vi "DO NOT DELETE acps project main ().vi"() -> ()   [LabVIEW 2026]
uses:
  <vilib>/DAQmx/write.llb/DAQmx Write (Counter Frequency 1Chan 1Samp).vi
  <vilib>/DAQmx/create/channels.llb/DAQmx Create Channel (CO-Pulse Generation-Frequency).vi
  <vilib>/DAQmx/configure/timing.llb/DAQmx Timing (Implicit).vi
  <vilib>/DAQmx/miscellaneous.llb/DAQmx Fill In Error Info.vi
panel:
  in  "stop 3":bool
  out "vibrating motor / LDR":bool
  out "smoke":bool
  out "temperature":dbl
  out "humidity":dbl
  in  "Tab Control":enum32{"Overview", "Detailed", "Advanced"}(tab)
  in  "Tol":dbl=10.0
  in  "Reset":bool
  out "Rotation":bool
  out "Jars Filled":dbl
  out "Weight":dbl(slide) scale=0.0..200.0
  out "State":dbl(ring) items=["0: Indexing / Seeking Jar"=0.0, "1: Reading Jar Colour"=1.0, "2: Stage 1 Filling"=2.0, "3: Stage 2 Dumping"=3.0, "4: Settle & Count"=4.0, "5: Clearing IR Beam"=5.0, "9: FAULT LATCHED!"=9.0]
  out "Total Weights Filled":dbl
  out "Target Weight":dbl
  out "Grains filling":bool
  in  "Red Weight":dbl=100.0
  in  "Green Weight":dbl=200.0
  in  "Blue Weight":dbl=300.0
  in  "Tare\nTare\nt\nT":bool
  in  "stop":bool
  out "IR":dbl
  out "LDR":dbl
  out "level":bool
  out "?":dbl[](array[numeric])
  out "Waveform Chart":dbl(graph)
  out "Faults":dbl
  out "IR":dynamicdata(graph)
  out "ldr":dynamicdata(graph)
  in  "K for":dbl=1046000.0
  out "Spread":dbl
  out "Vm":dbl
  out "Stable":bool
  out "Allow":dbl
  out "cmt":dbl
  out "v0":dbl
  out "done":dbl
  in  "stop 2":bool
  out "max value for colour sensor":dbl(graph)
  out "col":i32
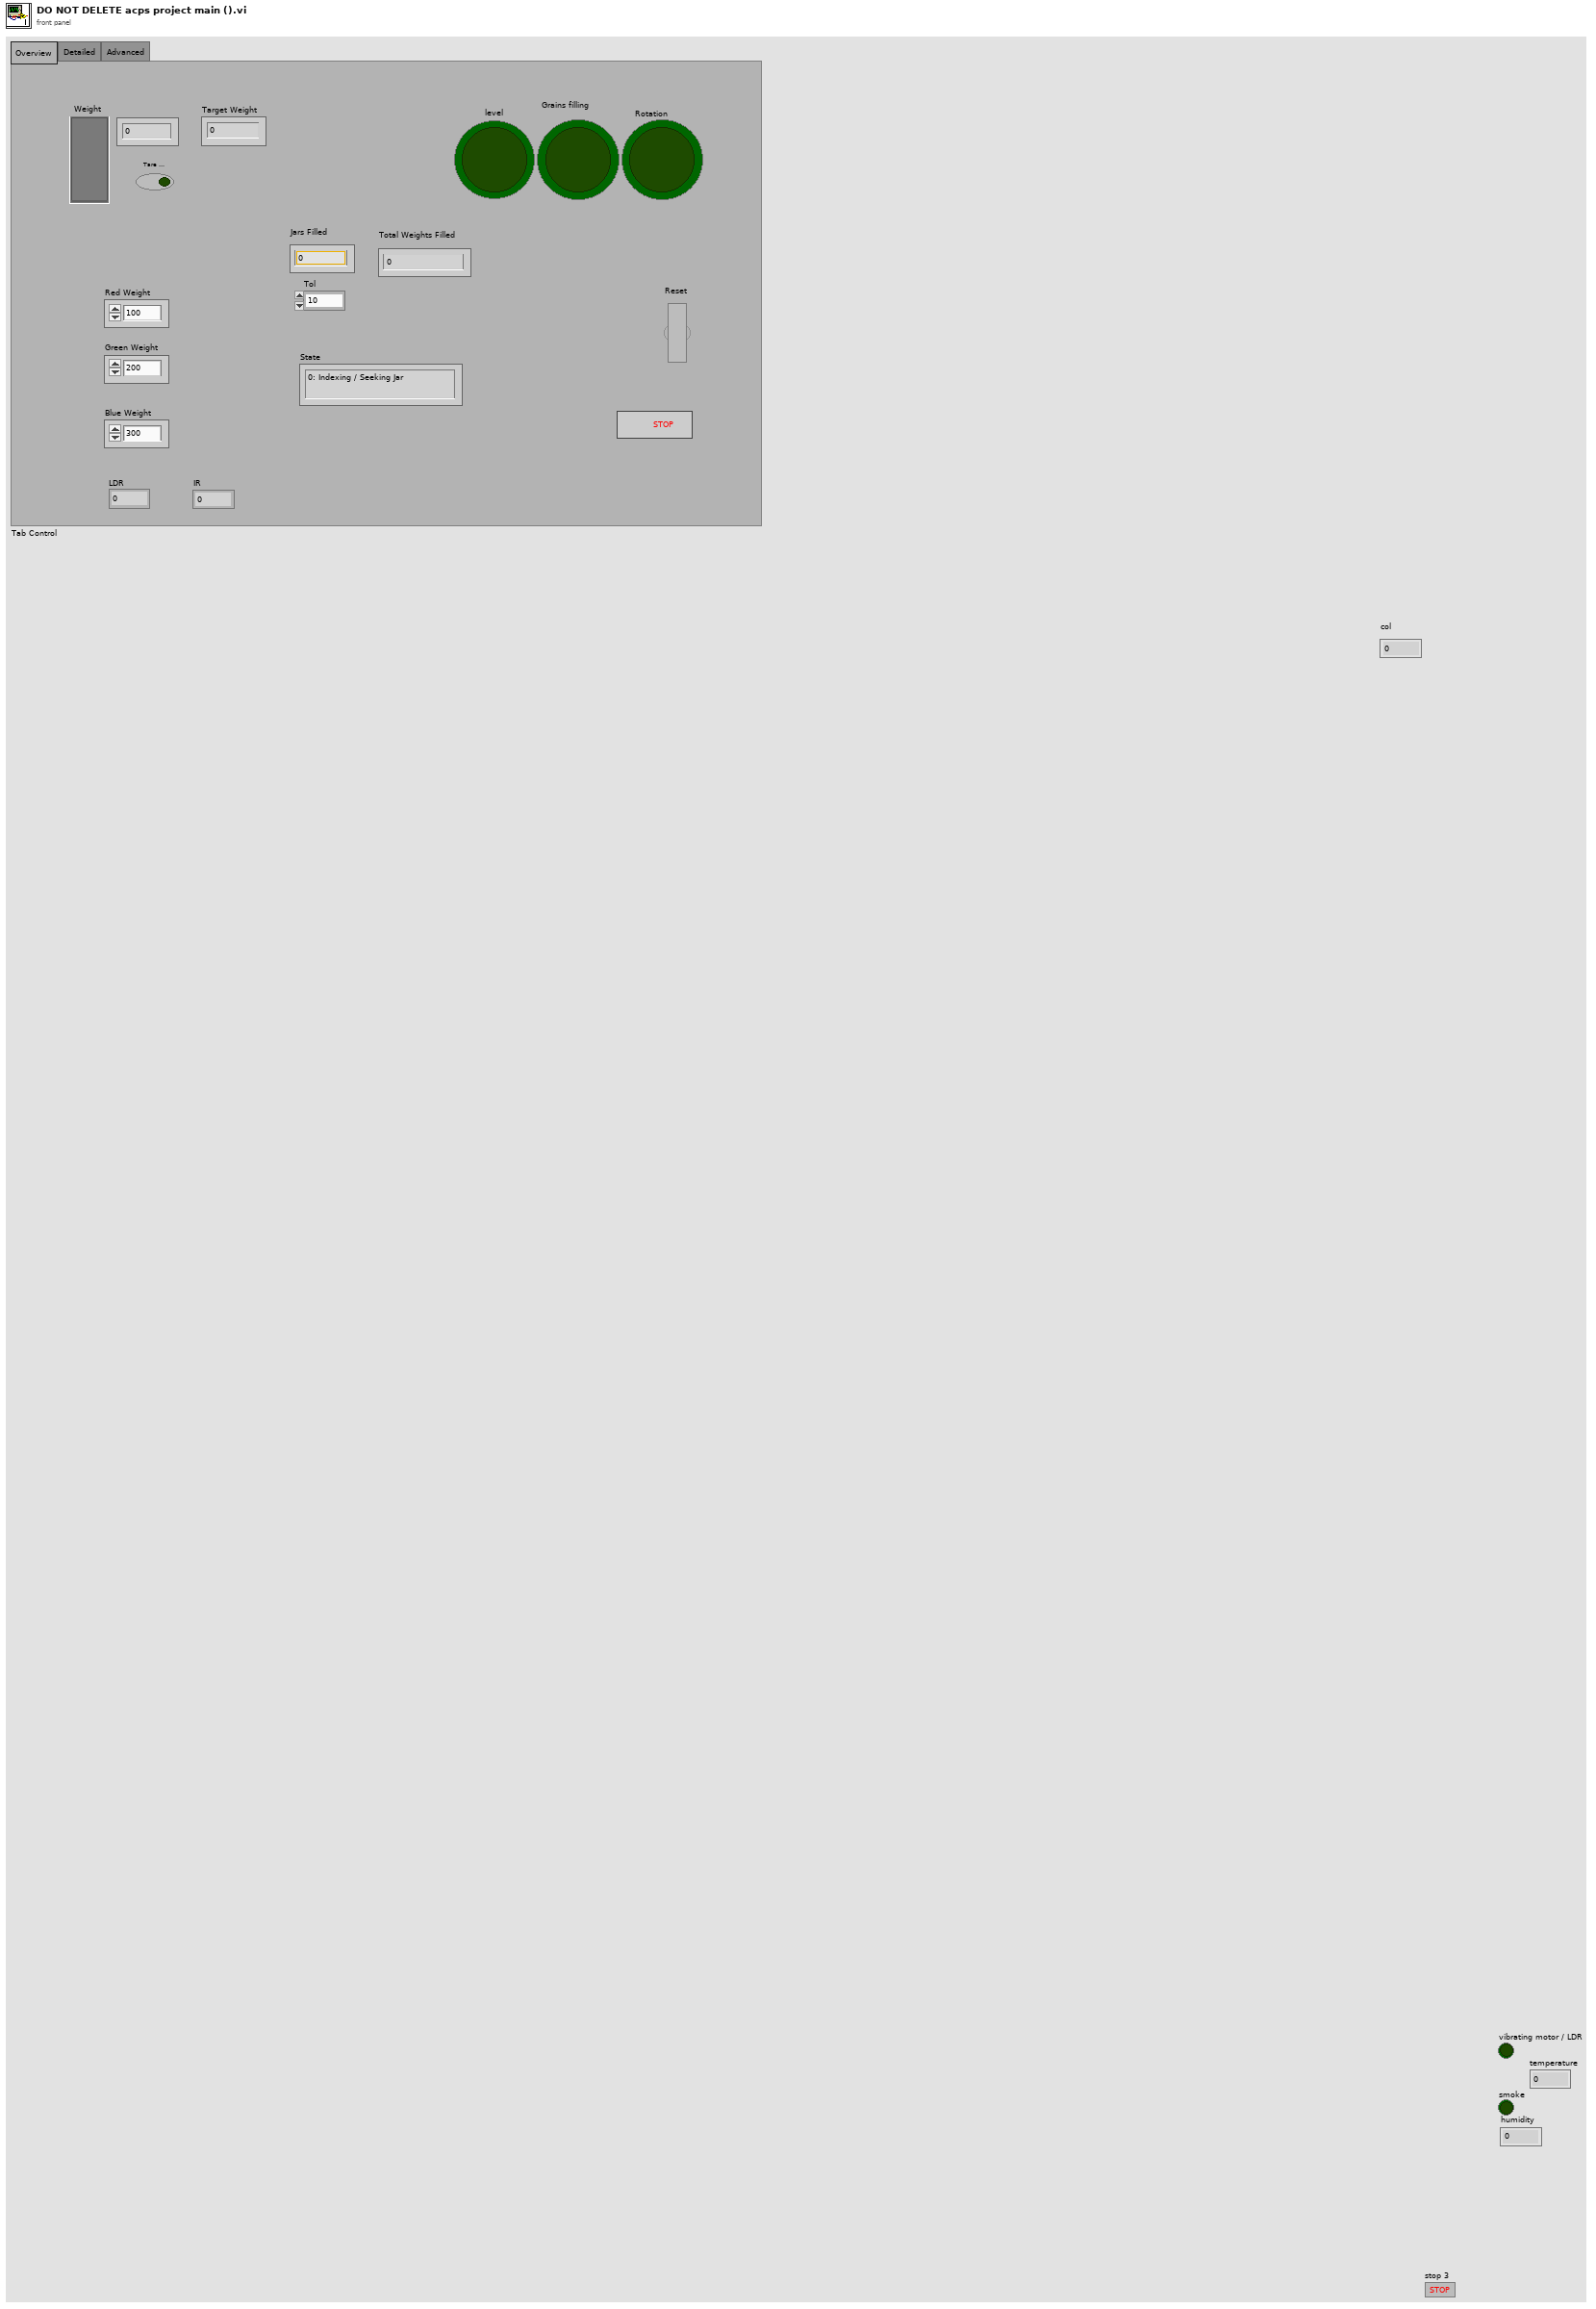
[diagram p1: front panel]
types:
  T1 = cluster{"LDR/Vibration ip":bool, "weight":dbl, "colour":i32}
  T2 = cluster{"vibrating motor / LDR":bool, "level sensor":bool, "Smoke/Fire":bool, "temperature":dbl, "humidity":dbl}
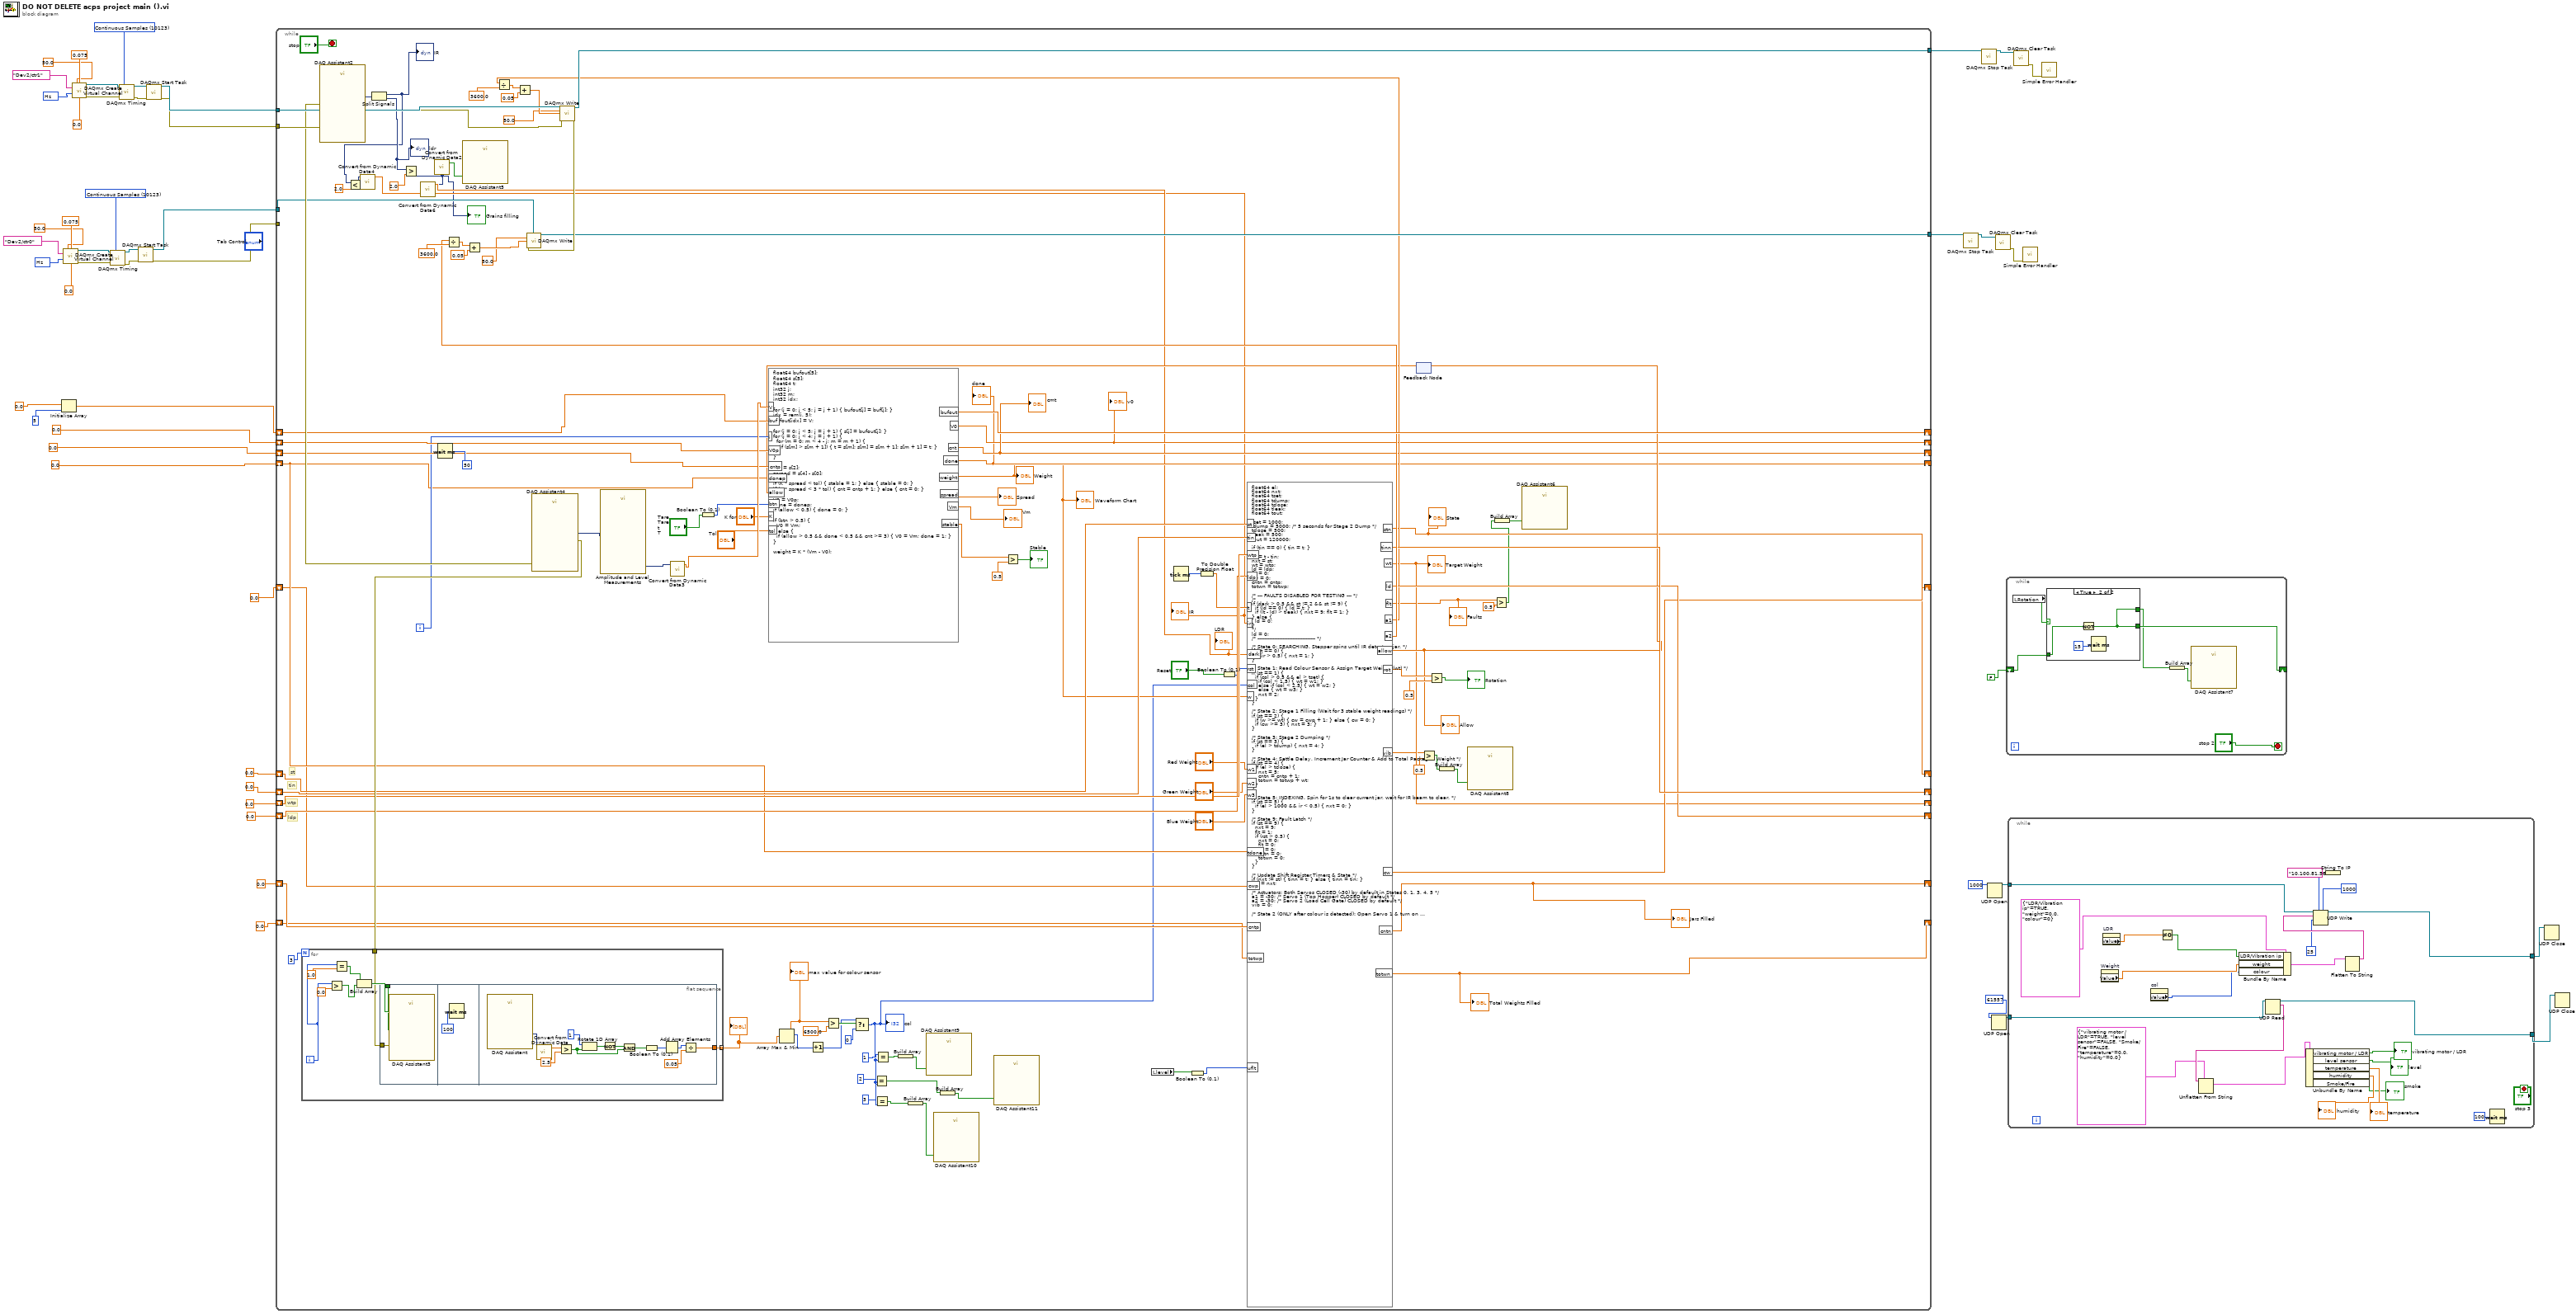
[diagram p0: block diagram]
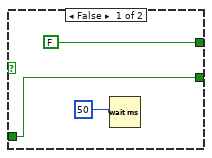
[diagram p2: hidden frame]
diagram:
  w25 = 10123 items=["Finite Samples"=10178, "Continuous Samples"=10123, "Hardware Timed Single Point"=12522] ("sample mode")
  w30 = 10373 items=["Hz"=10373] ("units")
  w45 = 10123 items=["Finite Samples"=10178, "Continuous Samples"=10123, "Hardware Timed Single Point"=12522] ("sample mode")
  w50 = 10373 items=["Hz"=10373] ("units")
  n1 = Initialize Array(0.0 ("element"), 5 ("dimension size")) -> (w10:dbl[])
  n2 = call-poly <vilib>:"DAQmx Create Virtual Channel.vi"("frequency"=50.0, "duty cycle"=0.075, "counter"=tag "Dev2/ctr0", "units"=w30, "initial delay"=0.0) -> ("task out"=w24:refnum<k21>, "error out"=w22:errorcluster)  [unwired: 9 in]
  n3 = call-poly <vilib>:"DAQmx Create Virtual Channel.vi"("frequency"=50.0, "duty cycle"=0.075, "counter"=tag "Dev2/ctr1", "units"=w50, "initial delay"=0.0) -> ("task out"=w44:refnum<k21>, "error out"=w41:errorcluster)  [unwired: 9 in]
  n4 = call-poly <vilib>:"DAQmx Timing.vi"("task/channels in"=w24, "sample mode"=w25, "error in"=w22) -> ("task out"=w23:refnum<k21>, "error out"=w21:errorcluster)  [unwired: 11 in]
  n5 = call-poly <vilib>:"DAQmx Timing.vi"("task/channels in"=w44, "sample mode"=w45, "error in"=w41) -> ("task out"=w43:refnum<k21>, "error out"=w40:errorcluster)  [unwired: 11 in]
  n6 = call <vilib>:"DAQmx Start Task.vi"("task/channels in"=w23, "error in"=w21) -> ("task out"=w20:refnum<k21>, "error out"=w19:errorcluster)  [unwired: 12 in]
  n7 = call <vilib>:"DAQmx Start Task.vi"("task/channels in"=w43, "error in"=w40) -> ("task out"=w42:refnum<k21>, "error out"=w39:errorcluster)  [unwired: 12 in]
  n8 = while {
    tunnel: w42 -> [w154]
    tunnel: w39 -> [w151]
    tunnel: [w149] -> w38
    shift-right: [w128] -> _
    shift-left: w10 -> [w137]
    shift-right: [w91] -> _
    shift-left: 0.0 ("element") -> [w90]
    shift-right: [w92] -> _
    shift-left: 0.0 ("element") -> [w136]
    shift-right: [w93] -> _
    shift-left: 0.0 ("element") -> [w135]
    tunnel: w20 -> [w122]
    tunnel: w19 -> [_]
    tunnel: [w120] -> w16
    shift-right: [w76] -> _
    shift-left: 0.0 -> [w113]
    shift-right: [w109] -> _
    shift-left: 0.0 -> [w112]
    shift-right: [w77] -> _
    shift-left: 0.0 -> [w111]
    shift-right: [w108] -> _
    shift-left: 0.0 -> [w110]
    shift-right: [w88] -> _
    shift-left: 0.0 -> [w89]
    shift-right: [w75] -> _
    shift-left: 0.0 -> [w83]
    shift-right: [w65] -> _
    shift-left: 0.0 -> [w66]
    i -> [w129]
    stop <- "stop" stop-if-true
    # "ldp"
    # "wtp"
    # "tin"
    # "st"
    n9 = call "DAQ Assistant2"() -> ("data"=w147:dynamicdata, "error out"=w145:errorcluster)  [unwired: 17 in, 1 out]
    n10 = Split Signals(w147) -> (w86:dynamicdata, w100:dynamicdata)  [unwired: 2 in]
    "IR" <- w86
    "ldr" <- w100
    n11 = Less?(x=w86, y=2.0) -> (x < y?=w85:dynamicdata)
    n12 = call "Convert from Dynamic Data4"("Dynamic Data Type"=w85) -> ("Scalar"=w79:dbl)  [unwired: 3 in]
    "IR" <- w79
    n13 = Greater?(x=w100, y=2.0) -> (0:w63:dynamicdata)
    "Grains filling" <- w63
    n14 = call "Convert from Dynamic Data6"("Dynamic Data Type"=w63) -> ("Scalar"=w80:dbl)  [unwired: 3 in]
    "LDR" <- w80
    n15 = call "Convert from Dynamic Data2"("Dynamic Data Type"=w63) -> ("Array"=w64:bool[])  [unwired: 3 in]
    n16 = Wait (ms)(milliseconds to wait=u32 50) -> ()  [unwired: 1 out]
    n17 = call "DAQ Assistant5"("data"=w64) -> ()  [unwired: 17 in, 2 out]
    n18 = call "DAQ Assistant4"("error in"=w145) -> ("data"=w144:dynamicdata, "error out"=w142:errorcluster)  [unwired: 16 in, 1 out]
    n19 = for {
      N: 3 -> [_]
      tunnel: [w160] -> w118 mode=indexing
      tunnel: w142 -> [w159]
      i -> [w164]
      n20 = Greater?(x=w164, y=0.0) -> (0:w162:bool)
      n21 = Equal?(x=w164, y=1.0) -> (x = y?=w163:bool)
      n22 = Build Array(w163, w162) -> (w161:bool[])
      n23 = flat-sequence {
        tunnel: w161 -> [w168]
        tunnel: w159 -> [w167]
        tunnel: [w171] -> w160
        frame #0 {
          n24 = call "DAQ Assistant3"("data"=w168, "error in"=w167) -> ()  [unwired: 16 in, 2 out]
        }
        frame #1 {
          n25 = Wait (ms)(milliseconds to wait=u32 100) -> ()  [unwired: 1 out]
        }
        frame #2 {
          n26 = call "DAQ Assistant"() -> ("data"=w181:dynamicdata)  [unwired: 17 in, 2 out]
          n27 = call "Convert from Dynamic Data"("Dynamic Data Type"=w181) -> ("Array"=w180:dbl[])  [unwired: 3 in]
          n28 = Greater?(x=w180, y=2.5) -> (0:w176:bool[])
          n29 = Rotate 1D Array(1:w176, 2:1 ("n")) -> (0:w178:bool[])
          n30 = Not(x=w178) -> (.not. x?=w177:bool[])
          n31 = And(x=w177, y=w176) -> (x .and. y?=w175:bool[])
          n32 = Boolean To (0,1)(Boolean=w175) -> (0, 1=w174:i16[])
          n33 = Add Array Elements(numeric array=w174) -> (sum=w173:i16)
          n34 = Divide(x=w173, y=0.05) -> (x/y=w171:dbl)
        }
      }
    }
    "?" <- w118
    n35 = call "Amplitude and Level Measurements"("Signals"=w144) -> ("Mean (DC)"=w143:dynamicdata)  [unwired: 13 in, 1 out]
    n36 = call "Convert from Dynamic Data3"("Dynamic Data Type"=w143) -> ("Scalar"=w141:dbl)  [unwired: 3 in]
    n37 = Boolean To (0,1)(Boolean="Tare\nTare\nt\nT") -> (0, 1=w138:i16)
    n38 = Array Max & Min(array=w118) -> (max value=w81:dbl, max index (indices)=w117:i32)  [unwired: 2 out]
    "max value for colour sensor" <- w81
    n39 = Increment(x=w117) -> (x+1=w116:i32)
    n40 = Greater?(x=w81, y=6500.0) -> (0:w119:bool)
    n41 = Select(t=w116, s=w119, f=0) -> (s? t:f=w59:i32)
    "col" <- w59
    n42 = Equal?(x=2, y=w59) -> (x = y?=w52:bool)
    n43 = Equal?(x=3, y=w59) -> (x = y?=w54:bool)
    n44 = Equal?(x=1, y=w59) -> (x = y?=w56:bool)
    n45 = Build Array(w56) -> (w55:bool[])
    n46 = Build Array(w54) -> (w53:bool[])
    n47 = call "DAQ Assistant9"("data"=w55) -> ()  [unwired: 17 in, 2 out]
    n48 = call "DAQ Assistant10"("data"=w53) -> ()  [unwired: 17 in, 2 out]
    n49 = Build Array(w52) -> (w51:bool[])
    n50 = call "DAQ Assistant11"("data"=w51) -> ()  [unwired: 17 in, 2 out]
    n51 = local read "level"() -> (w62:bool)
    n52 = Tick Count (ms)() -> (millisecond timer value=w107:u32)
    n53 = Boolean To (0,1)(Boolean=w62) -> (0, 1=w61:i16)
    n54 = To Double Precision Float(number=w107) -> (double precision float=w106:dbl)
    n55 = Boolean To (0,1)(Boolean="Reset") -> (0, 1=w104:i16)
    n56 = feedback #1() -> (w97:dbl)  [unwired: 1 in]
    n57 = formula code="float64 bufout[5];\nfloat64 s[5];\nfloat64 t;\nint32 j;\nint32 m;\nint32 idx;\n\nfor (j = 0; j < 5; j = j + 1) { bufout[j] = buf[j]; }\nidx = rem(i, 5);\nbufout[idx] = V;\n\nfor (j = 0; j < 5; j = j + 1) { s[j] = bufout[j]; }\nfor (j = 0; j < 4; j = j + 1) {\n  for (m = 0; m < 4 - j; m = m + 1) {\n    if (s[m] > s[m + 1]) { t = s[m]; s[m] = s[m + 1]; s[m + 1] = t; }\n  }\n}\n\nVm = s[2];\nspread = s[4] - s[0];\n\nif (K * spread < tol) { stable = 1; } else { stable = 0; }\nif (K * spread < 3 * tol) { cnt = cntp + 1; } else { cnt = 0; }\n\nV0 = V0p;\ndone = donep;\nif (allow < 0.5) { done = 0; }\n\nif (btn > 0.5) {\n  V0 = Vm;\n} else {\n  if (allow > 0.5 && done < 0.5 && cnt >= 3) { V0 = Vm; done = 1; }\n}\n\nweight = K * (Vm - V0);"("V"=w141, "buf"=w137, "i"=w129, "V0p"=w136, "cntp"=w135, "donep"=w90, "allow"=w97, "btn"=w138, "K"="K for", "tol"="Tol") -> ("bufout"=w128:dbl[], "V0"=w92:dbl, "cnt"=w93:dbl, "done"=w91:dbl, "weight"=w78:dbl, "spread"=→"Spread":dbl, "Vm"=→"Vm":dbl, "stable"=w99:dbl)
    "Weight" <- w78
    "Waveform Chart" <- w78
    "cmt" <- w93
    "v0" <- w92
    "done" <- w91
    n58 = Greater?(x=w99, y=0.5) -> (0:→"Stable":bool)
    n59 = formula code="float64 el;\nfloat64 nxt;\nfloat64 tset;\nfloat64 tdump;\nfloat64 tclose;\nfloat64 tleak;\nfloat64 tout;\n\ntset = 1000;\ntdump = 5000; /* 5 seconds for Stage 2 Dump */\ntclose = 500;\ntleak = 500;\ntout = 120000;\n\nif (tin == 0) { tin = t; }\n\nel = t - tin;\nnxt = st;\nwt = wtp;\nld = ldp;\nflt = 0;\ncw = 0;\ncntn = cntp;\ntotwn = totwp;\n\n/* --- FAULTS DISABLED FOR TESTING --- */\n/*\nif (dark > 0.5 && st != 2 && st != 9) {\n  if (ld == 0) { ld = t; }\n  if ((t - ld) > tleak) { nxt = 9; flt = 1; }\n} else {\n  ld = 0;\n}\n*/\nld = 0;\n/* ----------------------------------- */\n\n/* State 0: SEARCHING. Stepper spins until IR detects a jar. */\nif (st == 0) {\n  if (ir > 0.5) { nxt = 1; }\n}\n\n/* State 1: Read Colour Sensor & Assign Target Weight (wt) */\nif (st == 1) {\n  if (col > 0.5 && el > tset) {\n    if (col < 1.5) { wt = w1; } \n    else if (col < 2.5) { wt = w2; } \n    else { wt = w3; }\n    nxt = 2;\n  }\n}\n\n/* State 2: Stage 1 Filling (Wait for 3 stable weight readings) */\nif (st == 2) {\n  if (w >= wt) { cw = cwp + 1; } else { cw = 0; }\n  if (cw >= 3) { nxt = 3; }\n}\n\n/* State 3: Stage 2 Dumping */\nif (st == 3) {\n  if (el > tdump) { nxt = 4; }\n}\n\n/* State 4: Settle Delay, Increment Jar Counter & Add to Total Packaged Weight */\nif (st == 4) {\n  if (el > tclose) { \n    nxt = 5; \n    cntn = cntp + 1; \n    totwn = totwp + wt; \n  }\n}\n\n/* State 5: INDEXING. Spin for 1s to clear current jar, wait for IR beam to clear. */\nif (st == 5) {\n  if (el > 1000 && ir < 0.5) { nxt = 0; }\n}\n\n/* State 9: Fault Latch */\nif (st == 9) {\n  nxt = 9;\n  flt = 1; \n  if (rst > 0.5) { \n    nxt = 0; \n    flt = 0; \n    ld = 0; \n    cntn = 0; \n    totwn = 0; \n  }\n}\n\n/* Update Shift Register Timers & State */\nif (nxt != st) { tinn = t; } else { tinn = tin; }\nstn = nxt;\n\n/* Actuators: Both Servos CLOSED (-30) by default in States 0, 1, 3, 4, 5 */\na1 = -30; /* Servo 1 (Top Hopper) CLOSED by default */\na2 = -30; /* Servo 2 (Load Cell Gate) CLOSED by default */\nvib = 0;\n\n/* State 2 (ONLY after colour is detected): Open Servo 1 & turn on Vibrator */\nif (nxt == 2) { \n  a1 = 180; \n  vib = 1; \n}\n\n/* State 3 (Dumping): Servo 1 stays CLOSED (-30), Servo 2 swings OPEN (180) */\nif (nxt == 3) { \n  a2 = 180; \n}\n\nrot = 0;\nif (nxt == 0 || nxt == 5) { rot = 1; }\n\n/* Tare / System Ready Flag - TARES IN BOTH STATE 0 AND STATE 4 */\nallow = 0;\nif (nxt == 0 || nxt == 4) { allow = 1; }"("st"=w113, "tin"=w112, "wtp"=w111, "ldp"=w110, "t"=w106, "ir"=w79, "dark"=w80, "rst"=w104, "col"=w59, "w"=w78, "w1"="Red Weight", "w2"="Green Weight", "w3"="Blue Weight", "tdone"=w90, "cwp"=w89, "cntp"=w83, "totwp"=w66, "uflt"=w61) -> ("stn"=w76:dbl, "tinn"=w109:dbl, "wt"=w77:dbl, "ld"=w108:dbl, "flt"=w74:dbl, "a1"=w98:dbl, "a2"=w114:dbl, "allow"=w94:dbl, "rot"=w96:dbl, "cw"=w88:dbl, "cntn"=w75:dbl, "vib"=w70:dbl, "totwn"=w65:dbl)
    "State" <- w76
    "Target Weight" <- w77
    "Faults" <- w74
    "Allow" <- w94
    "Jars Filled" <- w75
    "Total Weights Filled" <- w65
    n60 = Divide(x=w114, y=3600.0) -> (x/y=w126:dbl)
    n61 = Add(x=w126, y=0.05) -> (x+y=w124:dbl)
    n62 = Divide(x=w98, y=3600.0) -> (x/y=w156:dbl)
    n63 = Add(x=w156, y=0.05) -> (x+y=w153:dbl)
    n64 = call-poly <vilib>:"DAQmx Write.vi"("task/channels in"=w154, "frequency"=50.0, "duty cycle"=w153, "error in"=w151) -> ("task out"=w149:refnum<k21>, "error out"=w121:errorcluster)  [unwired: 9 in, 1 out]
    n65 = call-poly <vilib>:"DAQmx Write.vi"("task/channels in"=w122, "frequency"=50.0, "duty cycle"=w124, "error in"=w121) -> ("task out"=w120:refnum<k21>)  [unwired: 9 in, 2 out]
    n66 = feedback-in #1(w94) -> ()
    n67 = Greater?(x=w70, y=0.5) -> (0:w68:bool)
    n68 = Greater?(x=w96, y=0.5) -> (0:→"Rotation":bool)
    n69 = Build Array(w68) -> (w67:bool[])
    n70 = call "DAQ Assistant8"("data"=w67) -> ()  [unwired: 17 in, 2 out]
    n71 = Greater?(x=w74, y=0.5) -> (0:w71:bool)
    n72 = Build Array(w71) -> (w72:bool[])
    n73 = call "DAQ Assistant6"("data"=w72) -> ()  [unwired: 17 in, 2 out]
  }
  n74 = call <vilib>:"DAQmx Stop Task.vi"("task/channels in"=w16) -> ("task out"=w18:refnum<k21>)  [unwired: 13 in, 1 out]
  n75 = call <vilib>:"DAQmx Stop Task.vi"("task/channels in"=w38) -> ("task out"=w37:refnum<k21>)  [unwired: 13 in, 1 out]
  n76 = UDP Open(11:u16 1000 ("port")) -> (port=w3:refnum<k16>)  [unwired: 4 in, 2 out]
  n77 = UDP Open(11:u16 61557 ("port or service name")) -> (port=w4:refnum<k16>)  [unwired: 4 in, 2 out]
  n78 = call <vilib>:"DAQmx Clear Task.vi"("task in"=w18) -> ("error out"=w17:errorcluster)  [unwired: 14 in]
  n79 = while {
    shift-right: [w184] -> _
    shift-left: FALSE ("stop 2") -> [w185]
    stop <- "stop 2" stop-if-true
    n80 = local read "Rotation"() -> (w187:bool)
    n81 = case shown="True" w187 {
      tunnel: w185 -> [w190 w193]
      tunnel: [w190 w191] -> w184
      tunnel: [FALSE ("stop 2") w191] -> w183
      frame False {
        n82 = Wait (ms)(milliseconds to wait=u32 50) -> ()  [unwired: 1 out]
      }
      frame True {
        n83 = Not(x=w193) -> (.not. x?=w191:bool)
        n84 = Wait (ms)(milliseconds to wait=u32 15) -> ()  [unwired: 1 out]
      }
    }
    n85 = Build Array(w183) -> (w182:bool[])
    n86 = call "DAQ Assistant7"("data"=w182) -> ()  [unwired: 17 in, 2 out]
  }
  n87 = while {
    tunnel: w4 -> [w213]
    tunnel: w3 -> [w212]
    tunnel: [w211] -> w2
    tunnel: [w210] -> w1
    stop <- "stop 3" stop-if-true
    n88 = property on="Weight" class="Slide (strict)"() -> ("Value"=w199:dbl)  [unwired: 2 in, 2 out]
    n89 = property on="LDR" class="DigNum (strict)"() -> ("Value"=w196:dbl)  [unwired: 2 in, 2 out]
    n90 = property on="col" class="DigNum (strict)"() -> ("Value"=w198:i32)  [unwired: 2 in, 2 out]
    n91 = Not Equal To 0?(x=w196) -> (x != 0?=w195:bool)
    n92 = Bundle By Name(cluster=T1 {"LDR/Vibration ip"=TRUE, "weight"=0.0, "colour"=0}, "LDR/Vibration ip"=w195, "weight"=w199, "colour"=w198) -> (w201:T1)
    n93 = UDP Read(connection ID=w213) -> (data out=w209:string, 3:w211:refnum<k16>)  [unwired: 3 in, 3 out]
    n94 = Unflatten From String(type=T2 {"vibrating motor / LDR"=TRUE, "level sensor"=FALSE, "Smoke/Fire"=FALSE, "temperature"=0.0, "humidity"=0.0}, binary string=w209) -> (value=w207:T2)  [unwired: 3 in, 2 out]
    n95 = Unbundle By Name(w207) -> ("vibrating motor / LDR"=→"vibrating motor / LDR":bool, "level sensor"=→"level":bool, "temperature"=→"temperature":dbl, "humidity"=→"humidity":dbl, "Smoke/Fire"=→"smoke":bool)
    n96 = String To IP(1:"10.100.81.58" ("name")) -> (0:w217:u32)
    n97 = Flatten To String(anything=w201) -> (data string=w200:string)  [unwired: 3 in, 2 out]
    n98 = UDP Write(address=w217, port or service name=u16 1000, connection ID=w212, data in=w200, 9:25 ("timeout ms (25000)")) -> (3:w210:refnum<k16>)  [unwired: 1 in, 1 out]
    n99 = Wait (ms)(milliseconds to wait=u32 100) -> ()  [unwired: 1 out]
  }
  n100 = call <vilib>:"DAQmx Clear Task.vi"("task in"=w37) -> ("error out"=w36:errorcluster)  [unwired: 14 in]
  n101 = call <vilib>:"Simple Error Handler.vi"("error in (no error)"=w17) -> ()  [unwired: 4 in, 5 out]
  n102 = call <vilib>:"Simple Error Handler.vi"("error in (no error)"=w36) -> ()  [unwired: 4 in, 5 out]
  n103 = UDP Close(connection ID=w1) -> ()  [unwired: 1 in, 2 out]
  n104 = UDP Close(connection ID=w2) -> ()  [unwired: 1 in, 2 out]
